vi "Edit Value.vi"(6 "Action":T1, 8 "error in (no error)":errorcluster, 10 "New Val":dbl, 11 "Sample in":refnum<class "Sample.lvclass">) -> (0 "error out":errorcluster, 3 "Sample out":refnum<class "Sample.lvclass">)   [LabVIEW 2020, in "Metrics.lvlib" / "Sample.lvclass"]
uses:
  Sample.lvclass
  Edit Action.ctl
  Sample.lvclass/Sample.ctl
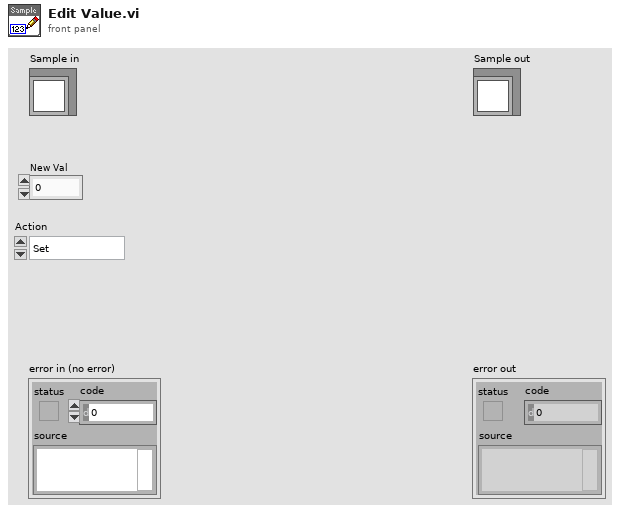
[diagram p1: front panel]
types:
  T1 = typedef "Metrics.lvlib/Sample.lvclass/Edit Action.ctl" = enum16{"Set", "Increment"}
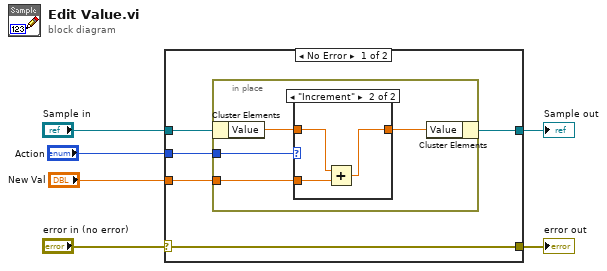
[diagram p0: block diagram]
diagram:
  n1 = case shown="No Error" "error in (no error)" {
    selector: "error in (no error)" -> [w11 w21]
    tunnel: [w11 w21] -> w5
    tunnel: [w8 w20] -> w3
    tunnel: "Sample in" -> [w10 w20]
    tunnel: "New Val" -> [w9 _]
    tunnel: "Action" -> [w7 _]
    frame No Error {
      n2 = in-place {
        in-place-border: w9 -> [w14]
        in-place-border: w7 -> [w12]
        n3 = in-place-cluster #1(w10) -> ("Value"=w15:dbl)
        n4 = case shown="\"Increment\"" w12 {
          tunnel: w15 -> [_ w19]
          tunnel: w14 -> [w16 w18]
          tunnel: [w16 w17] -> w13
          frame "Set", Default {
          }
          frame "Increment" {
            n5 = Add(x=w19, y=w18) -> (x+y=w17:dbl)
          }
        }
        n6 = in-place-cluster #1("Value"=w13) -> (w8:refnum<class "Sample.lvclass">)
      }
    }
    frame Error {
    }
  }
  "error out" <- w5
  "Sample out" <- w3
